vi "exp9_runner.vi"() -> ()   [LabVIEW 2020]
uses:
  Do Open Vi.vi
  Scripting Server.lvlib
  Do Add Subvi.vi
  Do Add To Selection.vi
  Do Enclose Selection.vi
  Do Save VI.vi
  add_subvi (Reply Payload)--cluster.ctl
  add_subvi Argument--cluster.ctl
  open_vi (Reply Payload)--cluster.ctl
  open_vi Argument--cluster.ctl
  add_to_selection (Reply Payload)--cluster.ctl
  add_to_selection Argument--cluster.ctl
  enclose_selection (Reply Payload)--cluster.ctl
  enclose_selection Argument--cluster.ctl
  save_vi (Reply Payload)--cluster.ctl
  save_vi Argument--cluster.ctl
panel:
  out "ErrCode5":dbl
  out "ErrCode4":dbl
  out "ErrCode3":dbl
  out "ErrCode2":dbl
  out "ErrCode1":dbl
  in  "ArgSave":T1
  in  "ArgEnc":T2
  in  "ArgSel":T3
  in  "ArgOpen":T4
  in  "add_subvi Argument":T5
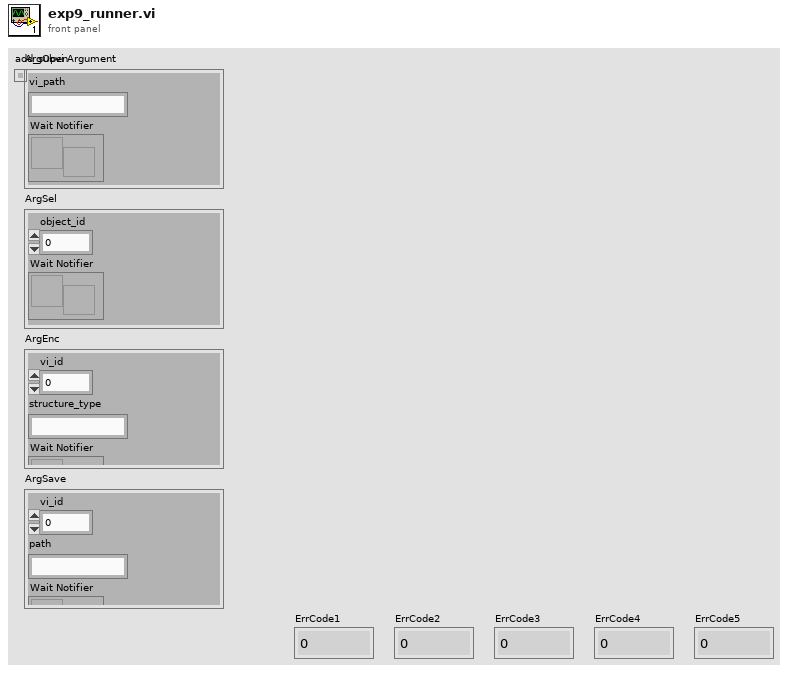
[diagram p1: front panel]
types:
  T1 = typedef "Scripting Server.lvlib/save_vi Argument--cluster.ctl" = cluster{"vi_id":i32, "path":string, "Wait Notifier":refnum<notifier>, "wait for reply":bool}
  T2 = typedef "Scripting Server.lvlib/enclose_selection Argument--cluster.ctl" = cluster{"vi_id":i32, "structure_type":string, "Wait Notifier":refnum<notifier>, "wait for reply":bool}
  T3 = typedef "Scripting Server.lvlib/add_to_selection Argument--cluster.ctl" = cluster{"object_id":i32, "Wait Notifier":refnum<notifier>, "wait for reply":bool, "vi_id":i32}
  T4 = typedef "Scripting Server.lvlib/open_vi Argument--cluster.ctl" = cluster{"vi_path":string, "Wait Notifier":refnum<notifier>, "wait for reply":bool}
  T5 = typedef "Scripting Server.lvlib/add_subvi Argument--cluster.ctl" = cluster{"diagram_id":i32, "subvi_path":string, "Wait Notifier":refnum<notifier>, "wait for reply":bool, "position_x":i32, "position_y":i32}
  T6 = typedef "Scripting Server.lvlib/Module Data--cluster.ctl" = cluster{"Status":string, "Current ID":i32, "References":variant, "Config Data":T7, "MCP id":i32, "Log":string}
  T7 = typedef "Scripting Server.lvlib/Config Data.ctl" = cluster{"Allowed Paths":string[]}
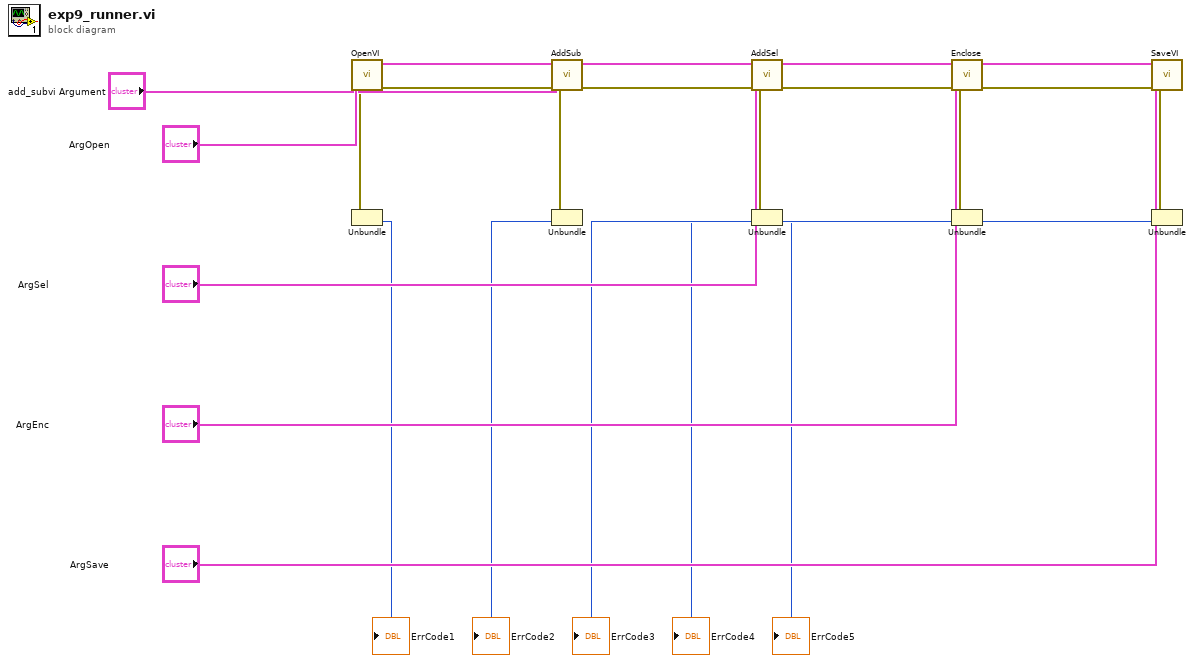
[diagram p0: block diagram]
diagram:
  n1 = call "OpenVI"("open_vi Argument"="ArgOpen") -> ("error out"=w10:errorcluster, "Data Cluster out"=w14:T6)  [unwired: 8 in, 1 out]
  n2 = Unbundle ("UB1")(w10) -> ("code"=→"ErrCode1":i32)  [unwired: 2 out]
  n3 = call "AddSub"("error in (no error)"=w10, "add_subvi Argument"="add_subvi Argument", "Data Cluster in"=w14) -> ("error out"=w9:errorcluster, "Data Cluster out"=w13:T6)  [unwired: 6 in, 1 out]
  n4 = Unbundle ("UB2")(w9) -> ("code"=→"ErrCode2":i32)  [unwired: 2 out]
  n5 = call "AddSel"("error in (no error)"=w9, "add_to_selection Argument"="ArgSel", "Data Cluster in"=w13) -> ("error out"=w8:errorcluster, "Data Cluster out"=w12:T6)  [unwired: 7 in]
  n6 = Unbundle ("UB3")(w8) -> ("code"=→"ErrCode3":i32)  [unwired: 2 out]
  n7 = call "Enclose"("error in (no error)"=w8, "enclose_selection Argument"="ArgEnc", "Data Cluster in"=w12) -> ("error out"=w7:errorcluster, "Data Cluster out"=w11:T6)  [unwired: 6 in, 1 out]
  n8 = Unbundle ("UB4")(w7) -> ("code"=→"ErrCode4":i32)  [unwired: 2 out]
  n9 = call "SaveVI"("error in (no error)"=w7, "save_vi Argument"="ArgSave", "Data Cluster in"=w11) -> ("error out"=w6:errorcluster)  [unwired: 6 in, 2 out]
  n10 = Unbundle ("UB5")(w6) -> ("code"=→"ErrCode5":i32)  [unwired: 2 out]
